vi "Read INI Key values.vi"(8 "error in (no error)":errorcluster, 9 "key":string, 10 "section":string, 11 "Path In":path) -> (0 "error out":errorcluster, 2 "value":string, 3 "Path Out":path)   [LabVIEW 2021]
uses:
  <vilib>/Utility/config.llb/Read Key (String).vi
  <vilib>/Utility/config.llb/NI_LVConfig.lvlib
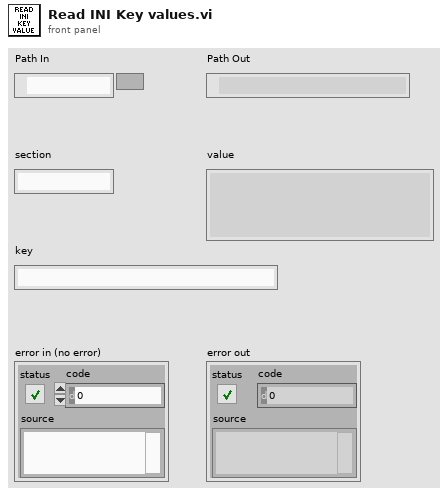
[diagram p1: front panel]
types:
  T1 = typedef "NI_LVConfig.lvlib/Config Data RefNum.ctl" = refnum<k1>
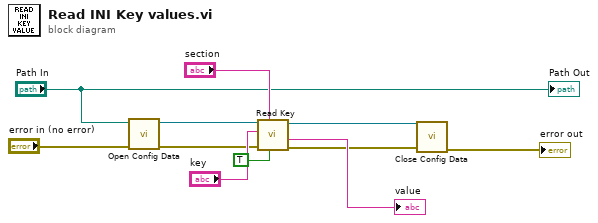
[diagram p0: block diagram]
diagram:
  n1 = call <vilib>:"Open Config Data.vi"("error in (no error)"="error in (no error)", "configuration file path"="Path In") -> ("error out"=w6:errorcluster, "refnum"=w5:T1)  [unwired: 7 in, 1 out]
  n2 = call-poly <vilib>:"Read Key.vi"("read raw string? (F)"=TRUE, "section"="section", "error in (no error)"=w6, "key"="key", "refnum"=w5) -> ("error out"=w9:errorcluster, "value"=→"value":string, "refnum out"=w8:T1)  [unwired: 3 in, 1 out]
  n3 = call <vilib>:"Close Config Data.vi"("error in (no error)"=w9, "refnum"=w8) -> ("error out"=→"error out":errorcluster)  [unwired: 8 in, 1 out]
  "Path Out" <- "Path In"
